vi "Open Block Diagram.vi"(8 "error in (no error)":errorcluster, 9 "Assertion Label":string, 10 "Call Chain":string[](array[string]), 11 "Basic Test Manager in":refnum<class "Basic Test Manager.lvclass">) -> (0 "error out":errorcluster, 3 "Basic Test Manager out":refnum<class "Basic Test Manager.lvclass">)   [LabVIEW 2020, in "Caraya.lvlib" / "Basic Test Manager.lvclass"]
uses:
  Basic Test Manager.lvclass
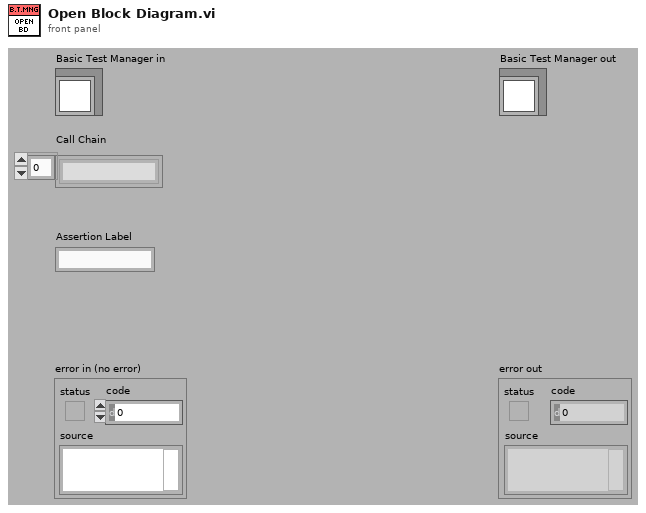
[diagram p1: front panel]
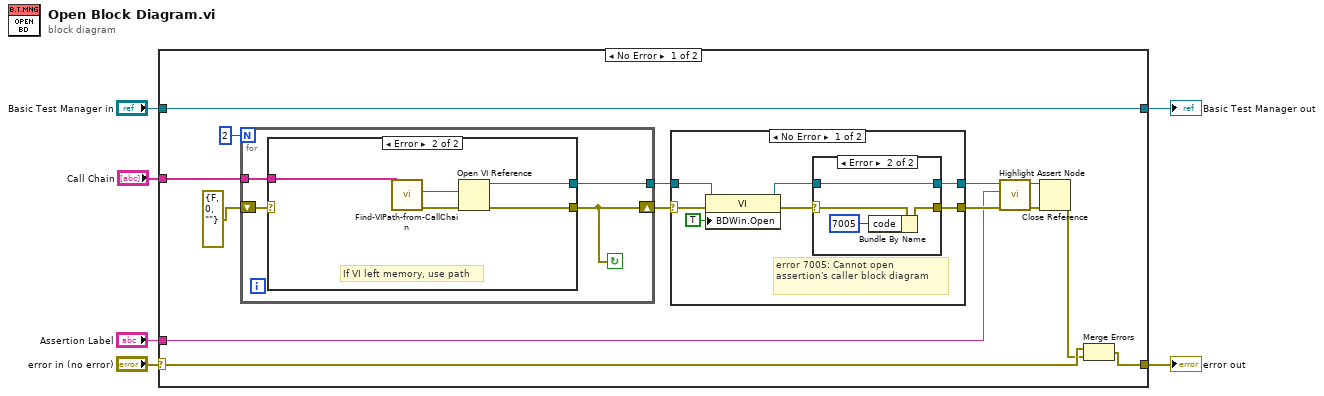
[diagram p0: block diagram]
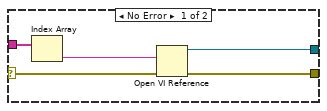
[diagram p4: hidden frame]
diagram:
  n1 = case shown="No Error" "error in (no error)" {
    selector: "error in (no error)" -> [w16 w51]
    tunnel: [w14 w51] -> w5
    tunnel: [w20 w50] -> w3
    tunnel: "Basic Test Manager in" -> [w20 w50]
    tunnel: "Call Chain" -> [w8 _]
    tunnel: "Assertion Label" -> [w9 _]
    frame No Error {
      n2 = for {
        N: 2 -> [_]
        tunnel: [w39] -> w19
        shift-right: [w38] -> w7
        shift-left: errorcluster {"status"=FALSE, "code"=0, "source"=""} ("error out") -> [w37]
        tunnel: w8 -> [w36]
        stop <- w38 continue-if-true
        n3 = case shown="Error" w37 {
          selector: w37 -> [w42 _]
          tunnel: [w44 w48] -> w39
          tunnel: [w43 w49] -> w38
          tunnel: w36 -> [w41 w46]
          frame No Error {
            n4 = Index Array(array=w41) -> (element=w40:string)  [unwired: 1 in]
            n5 = Open VI Reference(vi path=w40, error in (no error)=w42) -> (vi reference=w44:refnum<vi>, error out=w43:errorcluster)  [unwired: 4 in]
          }
          frame Error {
            # "If VI left memory, use path"
            n6 = call "Find-VIPath-from-CallChain.vi"("Call Chain"=w46) -> ("error out"=w47:errorcluster, "VI Path"=w45:path)  [unwired: 9 in]
            n7 = Open VI Reference(vi path=w45, error in (no error)=w47) -> (vi reference=w48:refnum<vi>, error out=w49:errorcluster)  [unwired: 4 in]
          }
        }
      }
      n8 = case shown="No Error" w7 {
        selector: w7 -> [w25 w35]
        tunnel: w19 -> [w27 w34]
        tunnel: [w22 w34] -> w13
        tunnel: [w23 w35] -> w11
        frame No Error {
          # "error 7005: Cannot open assertion's caller block diagram"
          n9 = property class="VI"(reference=w27, error in=w25, "BDWin.Open"=TRUE ("Block Diagram Window:Open")) -> (reference out=w21:refnum<vi>, error out=w24:errorcluster)
          n10 = case shown="Error" w24 {
            selector: w24 -> [w29 w33]
            tunnel: [w29 w31] -> w23
            tunnel: [w28 w30] -> w22
            tunnel: w21 -> [w28 w30]
            frame No Error {
            }
            frame Error {
              n11 = Bundle By Name(cluster=w33, "code"=7005) -> (w31:errorcluster)
            }
          }
        }
        frame Error {
        }
      }
      n12 = call "Highlight Assert Node.vi"("error in (no error)"=w11, "Assertion Label"=w9, "vi reference"=w13) -> ("error out"=w10:errorcluster, "vi reference  dup"=w12:refnum<vi>)  [unwired: 7 in]
      n13 = Close Reference(reference=w12, error in (no error)=w10) -> (error out=w15:errorcluster)
      n14 = Merge Errors(w16, w15) -> (w14:errorcluster)
    }
    frame Error {
    }
  }
  "error out" <- w5
  "Basic Test Manager out" <- w3
